vi "Base assingnment EXVI_MS.vi"(5 "BR all info":T11, 6 "Total assembly C":T6 {"Assembly Ratio 2" format="%#_3g"; "Assembly Ratio" format="%#_3g"}, 7 "BC1":cluster{"B region#":i32, "Date":string}, 8 "error in":errorcluster caption="エラー入力", 9 "Selected Raw D":T15, 10 "S New Info and MiN":T26={"Sample Sequence"="GATGATGATGATGATGAT", "Right Read MIN"=6, "Filter P"=0, "STD Type"=enum."Region", "Base Table"=[], "Selection"=enum."10kHz", "noise MAX"=3, "Sample name"=""} {"Base Table"."Value 3" format="%.2g"}, 11 "Filename Path":path) -> (0 "error out":errorcluster caption="エラー出力", 1 "GR data":T21, 2 "Data Histogram":T32(graph), 3 "Table cluster_B":T4, 4 "Ex info":T16)   [LabVIEW 2018]
panel:
  out "Assigned CP Profile plus":T1
  out "Assinged Signal Profile plus":T2
  out "Assigned Time Profile plus":T3
  out "LAP Table":string[][](table) caption="LCP Table"
  out "SOC cluster":T5
  out "Base N info":T7
  out "B Cluster":T8
  out "R std Level":dbl[](array[numeric])
  out "STD Type":enum16{"Region", "Each", "Fixed"}(ring)
  out "BR BL and STD info":T9
  out "BR info":T10
  out "BS Path":T12
  out "BNAL Path":T13
  out "LS Path":T14
  out "B region#":i32
  out "Date":string
  out "Pre File F_Name":string
  out "Base Ex Info":T17
  in  "Data Estimated Info":T18
  out "Base info":T19
  out "Filter P":i32
  out "CP Profile Table P":string[][](table) caption="CP Table"
  out "Time Profile Table P":string[][](table) caption="Time Table"
  out "Signal Profile Table P":string[][](table) caption="表"
  out "Level Composition":string[](array[string])
  out "A level":dbl[](array[numeric])
  out "Filename":string
  out "Time A Table AZ":string[](array[string])
  out "LTP Table":string[][](table) caption="L Time Table for plot"
  out "Filtered Current":dbl[](array[numeric])
  out "Change Point Array":T20
  out "CP Probability":dbl[][](array[numeric])
  out "Time Probability":dbl[][](array[numeric])
  out "Save CV":T22
  out "Table Tag":T23
  out "Table CV":T24
  out "Time A Table Tag":string[](array[string])
  out "CP A Tag AZ":string[](array[string])
  out "Color":u32[](array[numeric])
  out "ASM C":T25
  out "Signal Tag AZ":string[](array[string])
  out "Signal A Table Tag":string[](array[string])
  out "CP A Table Tag":string[](array[string])
  out "R Level":dbl[](array[numeric])
  out "Signal Profile Table":string[][](table) caption="Singla Profile Table"
  in  "Control":enum32{"Set P", "S", "CP", "T"}(tab)
  out "BS Table":string[][](table) caption="Singla Profile Table"
  out "CP Profile Table":string[][](table) caption="CP Table"
  out "Time Profile Table":string[][](table) caption="Time Table"
  in  "I-t":enum32{"Time", "CP", "Assembly", "Plot"}(tab)
  out "Time Graph":cluster{"time":dbl[], "current":dbl[]}[](graph)
  out "Time Graph Profile":cluster{"time":dbl[], dbl[]}[](graph)
  out "Label":T27
  out "CP Graph":cluster{i32[], dbl[]}[](graph)
  out "CP Graph Profile":cluster{i32[], dbl[]}[](graph)
  out "Label 2":T27
  out "std [ratio]":T28={"CP std (ratio)"=200.0, "P std (ratio)"=200.0} {"P std (ratio)" format="%#_3g"; "CP std (ratio)" format="%#_3g"}
  out "Long Assembly":bool[][](array[boolean])
  out "All assembly":bool[][](array[boolean])
  out "assembly C":T29
  out "Signal Number Histogram":cluster{"配列 2":i32[], "配列 5":dbl[]}[](graph)
  out "Right Read MIN":i32=4
  out "LSP Table":string[][](table) caption="Long Singla Profile Table"
  out "Cutted Sample Sequence":string
  out "Base Species (n)":i32
  out "Base (n)":i32
  out "SN [ratio]":T30
  out "Plot Graph":dbl[][](graph)
  out "LCP Table":string[][](table)
  out "F std [pA]":cluster{"CP std (pA)":dbl, "P std (pA)":dbl}={"CP std (pA)"=200.0, "P std (pA)"=200.0} {"P std (pA)" format="%#_13g"; "CP std (pA)" format="%#_13g"}
  out "Relative Data Array":dbl[](array[numeric])
  out "Base Composition":string[](array[string])
  out "Each Base Sequence Info":T31
  out "Sample Sequence":string="GATGATGATGAT"
  in  "time":dbl[](array[numeric])
  in  "current":dbl[](array[numeric])
  out "BS txt":dbl[][](array[numeric])
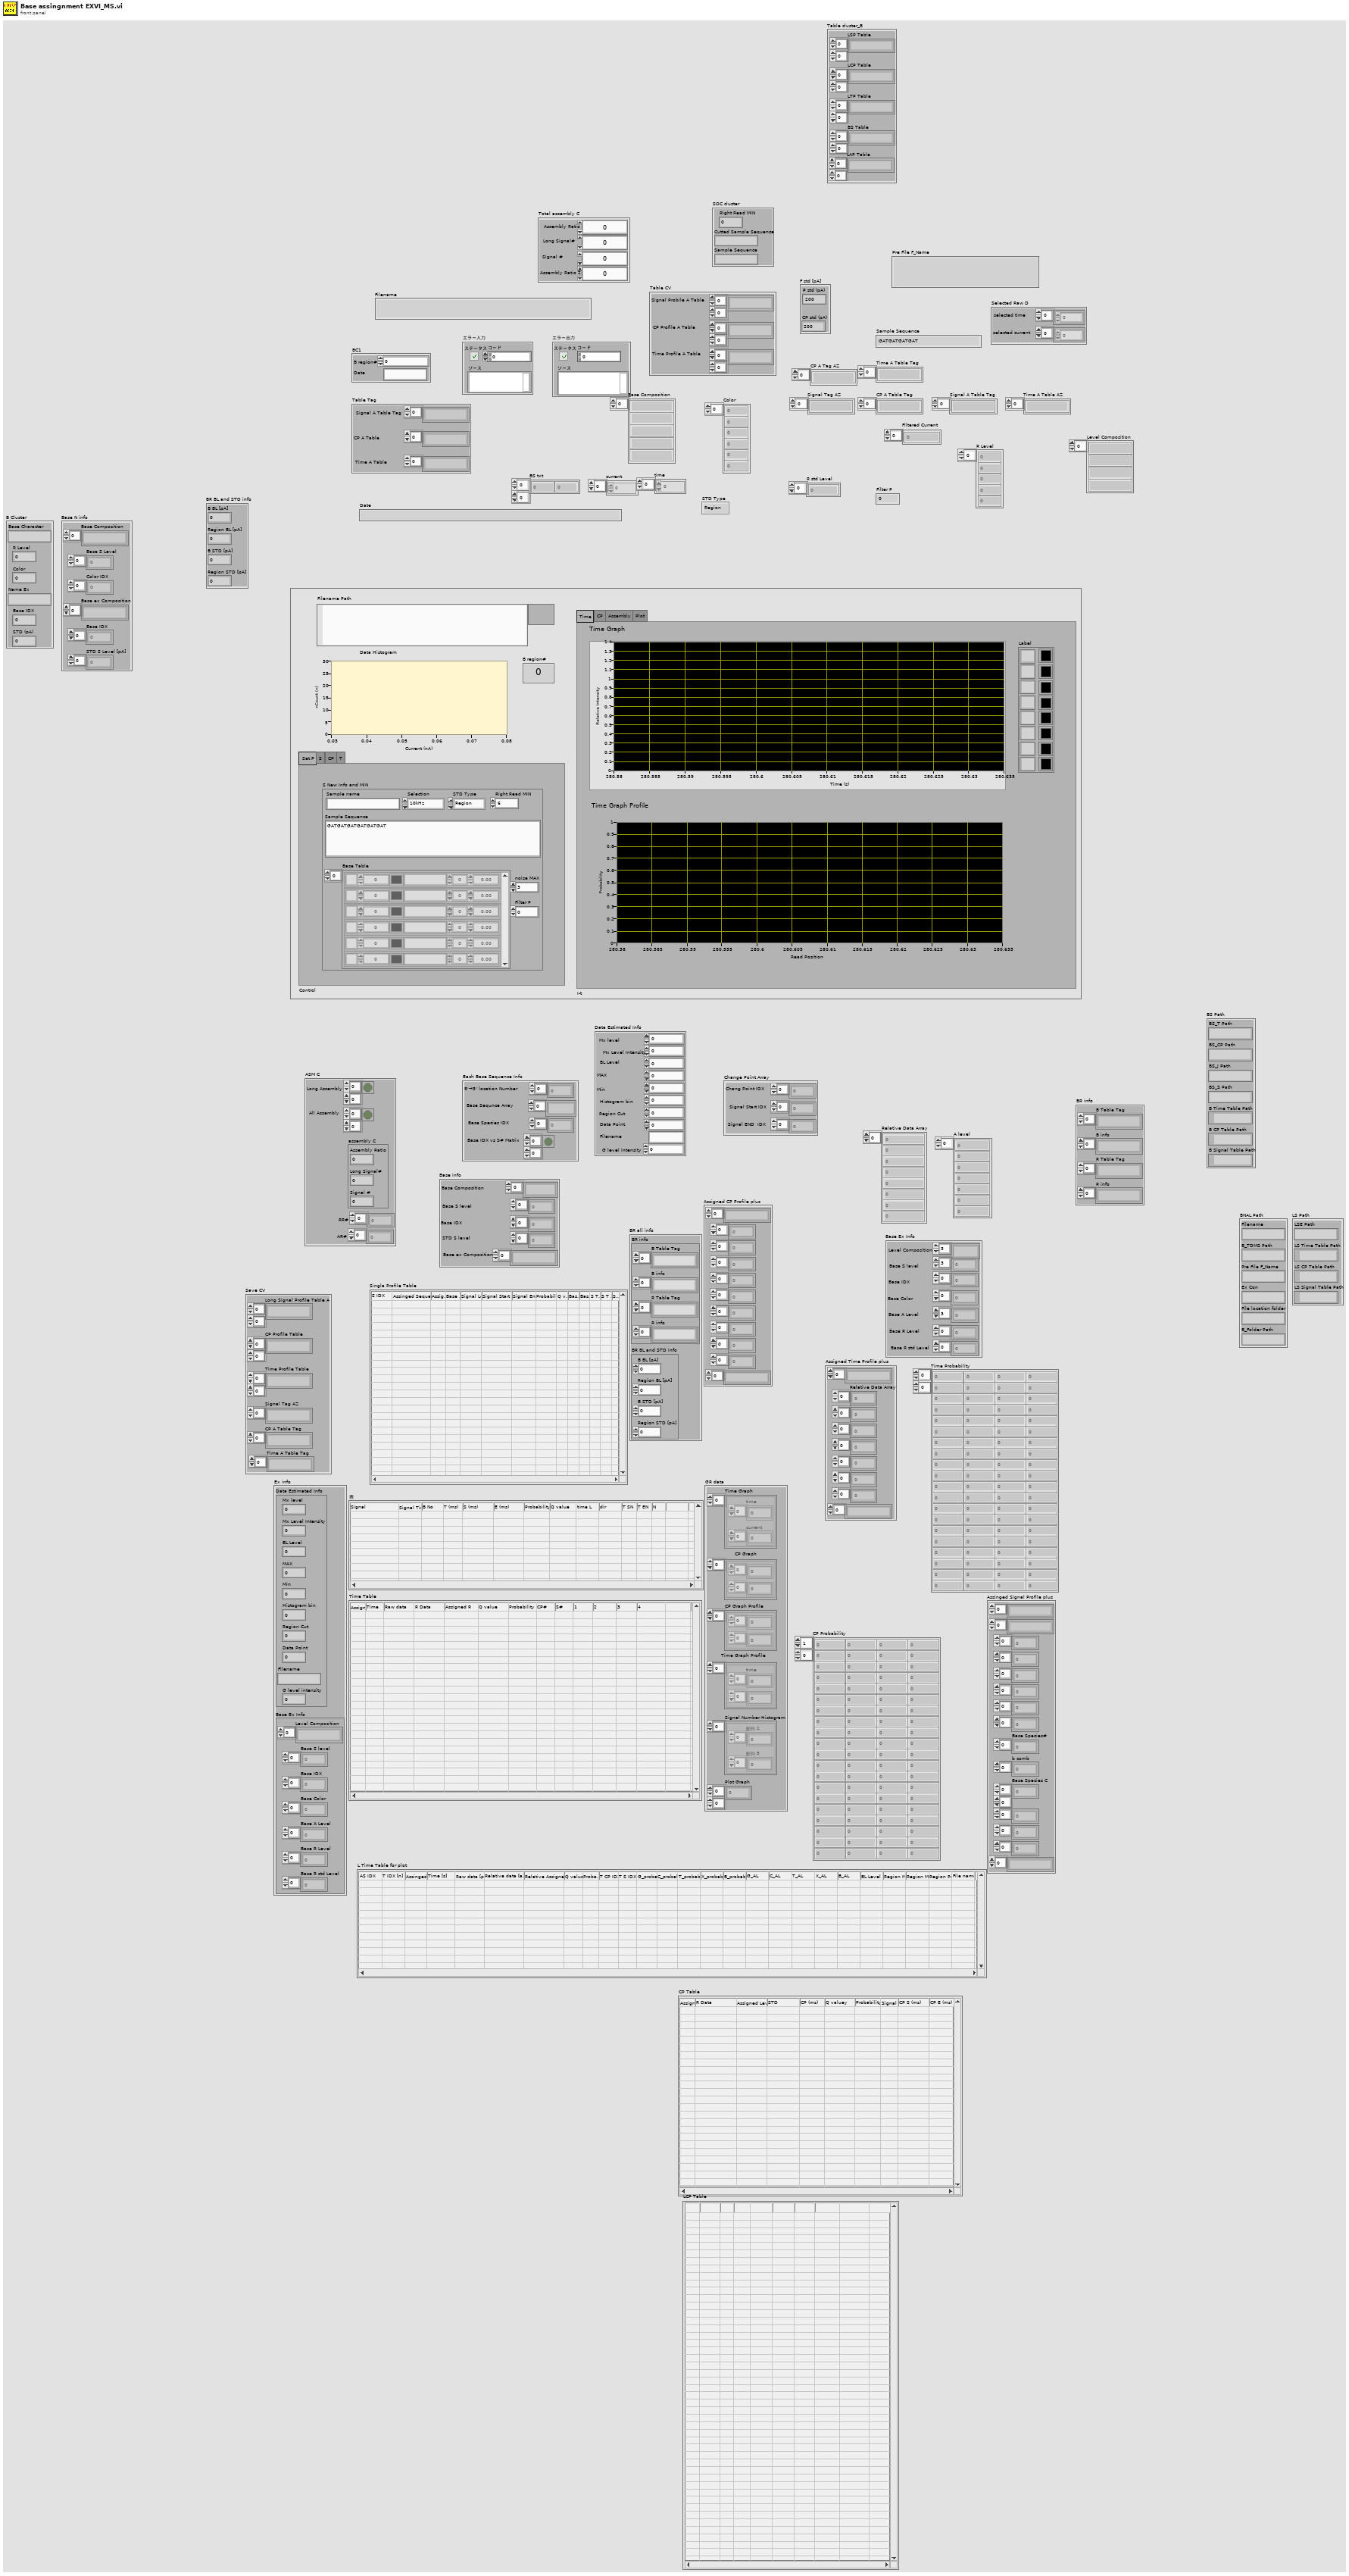
[diagram p1: front panel]
types:
  T1 = cluster{string[], dbl[], dbl[], dbl[], i32[], dbl[], dbl[], i32[], i32[], i32[], string[]}
  T2 = cluster{string[], string[], i32[], i32[], i32[], i32[], dbl[], dbl[], "Base Species#":i16[], "b comb":u32[], "Base Species C":i32[][], i32[], i32[], i32[], string[]}
  T3 = cluster{string[], "Relative Data Array":dbl[], dbl[], dbl[], dbl[], i32[], i32[], i32[], string[]}
  T4 = cluster{"LSP Table":string[][], "LCP Table":string[][], "LTP Table":string[][], "BS Table":string[][], "LAP Table":string[][]}
  T5 = cluster{"Right Read MIN":i32, "Cutted Sample Sequence":string, "Sample Sequence":string}
  T6 = cluster{"Assembly Ratio":dbl, "Long Signal#":i32, "Signal #":i32, "Assembly Ratio 2":dbl}
  T7 = cluster{"Base Composition":string[], "Base S Level":dbl[], "Color IDX":u32[], "Base ex Composition":string[], "Base IDX":i32[], "STD S Level [pA]":dbl[]}
  T8 = cluster{"Base Character":string, "R Level":dbl, "Color":u32, "Name Ex":string, "Base IDX":dbl, "STD (pA)":dbl}
  T9 = cluster{"B BL [pA]":dbl, "Region BL [pA]":dbl, "B STD [pA]":dbl, "Region STD [pA]":dbl}
  T10 = cluster{"B Table Tag":string[], "B info":string[], "R Table Tag":string[], "R info":string[]}
  T11 = cluster{"BR info":cluster{"B Table Tag":string[], "B info":string[], "R Table Tag":string[], "R info":string[]}, "BR BL and STD info":cluster{"B BL [pA]":dbl, "Region BL [pA]":dbl, "B STD [pA]":dbl, "Region STD [pA]":dbl}}
  T12 = cluster{"BS_T Path":string, "BS_CP Path":string, "BS_J Path":string, "BS_S Path":string, "B Time Table Path":path, "B CP Table Path":path, "B Signal Table Path":path}
  T13 = cluster{"Filename":string, "B_TDMS Path":string, "Pre File F_Name":string, "Ex Con":string, "File location folder":string, "B_Folder Path":string}
  T14 = cluster{"LSE Path":string, "LS Time Table Path":path, "LS CP Table Path":path, "LS Signal Table Path":path}
  T15 = cluster{"selected time":dbl[], "selected current":dbl[]}
  T16 = cluster{"Data Estimated Info":cluster{"Mx level":dbl, "Mx Level Intensity":dbl, "BL Level":dbl, "MAX":dbl, "Min":dbl, "Histogram bin":dbl, "Region Cut":dbl, "Data Point":i32, "Filename":string, "G level intensity":dbl}, "Base Ex Info":cluster{"Level Composition":string[], "Base S level":dbl[], "Base IDX":i32[], "Base Color":u32[], "Base A Level":dbl[], "Base R Level":dbl[], "Base R std Level":dbl[]}}
  T17 = cluster{"Level Composition":string[], "Base S level":dbl[], "Base IDX":i32[], "Base Color":u32[], "Base A Level":dbl[], "Base R Level":dbl[], "Base R std Level":dbl[]}
  T18 = cluster{"Mx level":dbl, "Mx Level Intensity":dbl, "BL Level":dbl, "MAX":dbl, "Min":dbl, "Histogram bin":dbl, "Region Cut":dbl, "Data Point":i32, "Filename":string, "G level intensity":dbl}
  T19 = cluster{"Base Composition":string[], "Base S level":dbl[], "Base IDX":i32[], "STD S level":dbl[], "Base ex Composition":string[]}
  T20 = cluster{"Chang Point IDX":i32[], "Signal Start IDX":i32[], "Signal END  IDX":i32[]}
  T21 = cluster{"Time Graph":cluster{"time":dbl[], "current":dbl[]}[], "CP Graph ":cluster{i32[], dbl[]}[], "CP Graph Profile":cluster{i32[], dbl[]}[], "Time Graph Profile":cluster{"time":dbl[], dbl[]}[], "Signal Number Histogram":cluster{"配列 2":i32[], "配列 5":dbl[]}[], "Plot Graph":dbl[][]}
  T22 = cluster{"Long Signal Profile Table A ":string[][], "CP Profile Table":string[][], "Time Profile Table":string[][], "Signal Tag AZ":string[], "CP A Table Tag":string[], "Time A Table Tag":string[]}
  T23 = cluster{"Signal A Table Tag":string[], "CP A Table":string[], "Time A Table":string[]}
  T24 = cluster{"Signal Probile A Table":string[][], "CP Profile A Table":string[][], "Time Profile A Table":string[][]}
  T25 = cluster{"Long Assembly":bool[][], "All Assembly":bool[][], "assembly C":cluster{"Assembly Ratio":dbl, "Long Signal#":i32, "Signal #":i32}, "RR#":i32[], "AR#":i32[]}
  T26 = cluster{"Sample Sequence":string, "Right Read MIN":i32, "Filter P":i32, "STD Type":enum16{"Region", "Each", "Fixed"}, "Base Table":cluster{"Name":string, "Value":dbl, "Color":u32, "Name 2":string, "Value 2":dbl, "Value 3":dbl}[], "Selection":enum16{"10kHz", "100kHz"}, "noise MAX":i32, "Sample name":string}
  T27 = cluster{"カラーボックス":u32, "カラーボックス 4":u32, "カラーボックス 2":u32, "カラーボックス 5":u32, "カラーボックス 3":u32, "カラーボックス 6":u32, "カラーボックス 7":u32, "カラーボックス 8":u32, "B0":string, "B1":string, "B2":string, "B3":string, "B4":string, "B5":string, "B6":string, "B7":string}
  T28 = cluster{"CP std (ratio)":dbl, "P std (ratio)":dbl}
  T29 = cluster{"Assembly Ratio":dbl, "Long Signal#":i32, "Signal #":i32}
  T30 = cluster{"CP S/N ratio":dbl, "T S/N ratio":dbl, "Mx Intensity level [pA]":dbl}
  T31 = cluster{"5'→3' location Number":i32[], "Base Sequnce Array":string[], "Base Species IDX":i32[], "Base IDX vs S# Matrix":bool[][]}
  T32 = cluster{"X Values":dbl[], "Histogram: h(x)":i32[]}
  T33 = cluster{"Name":string, "Value":dbl, "Color":u32, "Name 2":string, "Value 2":dbl, "Value 3":dbl}[]
  T34 = cluster{"B S/N ratio":dbl, "R S/N ratio":dbl, "Mx Intensity level [pA]":dbl}
  T35 = cluster{"CP std [ratio]":dbl, "T std [ratio]":dbl}
  T36 = cluster{"Value":cluster{"Mx level":dbl, "Mx Level Intensity":dbl, "BL Level":dbl, "MAX":dbl, "Min":dbl, "Histogram bin":dbl, "Region Cut":dbl, "Data Point":i32, "Filename":string, "G level intensity":dbl}, "Base Ex Info":cluster{"Level Composition":string[], "Base S level":dbl[], "Base IDX":i32[], "Base Color":u32[], "Base A Level":dbl[], "Base R Level":dbl[], "Base R std Level":dbl[]}}
  T37 = cluster{"Value":string[][], "Value":string[][], "Value":string[][]}
  T38 = cluster{"Value":i32, "Value":string, "Value":string}
  T39 = cluster{"Signal Tag A":string[], "L Signal Tag A":string[]}
  T40 = cluster{"LAP_Table_Tag":string[], "LAP_Table":string[][]}
  T41 = cluster{"Value":string[][], "Value":string[][], "Value":string[][], "Value":string[][], "Value":string[][]}
  T42 = cluster{"Value":cluster{"time":dbl[], "current":dbl[]}[], "Value":cluster{i32[], dbl[]}[], "Value":cluster{i32[], dbl[]}[], "Value":cluster{"time":dbl[], dbl[]}[], "Value":cluster{"配列 2":i32[], "配列 5":dbl[]}[], "Value":dbl[][]}
  T43 = cluster{"Value":string[][], "Value":string[][], "Value":string[][], "Value":string[], "Value":string[], "Value":string[]}
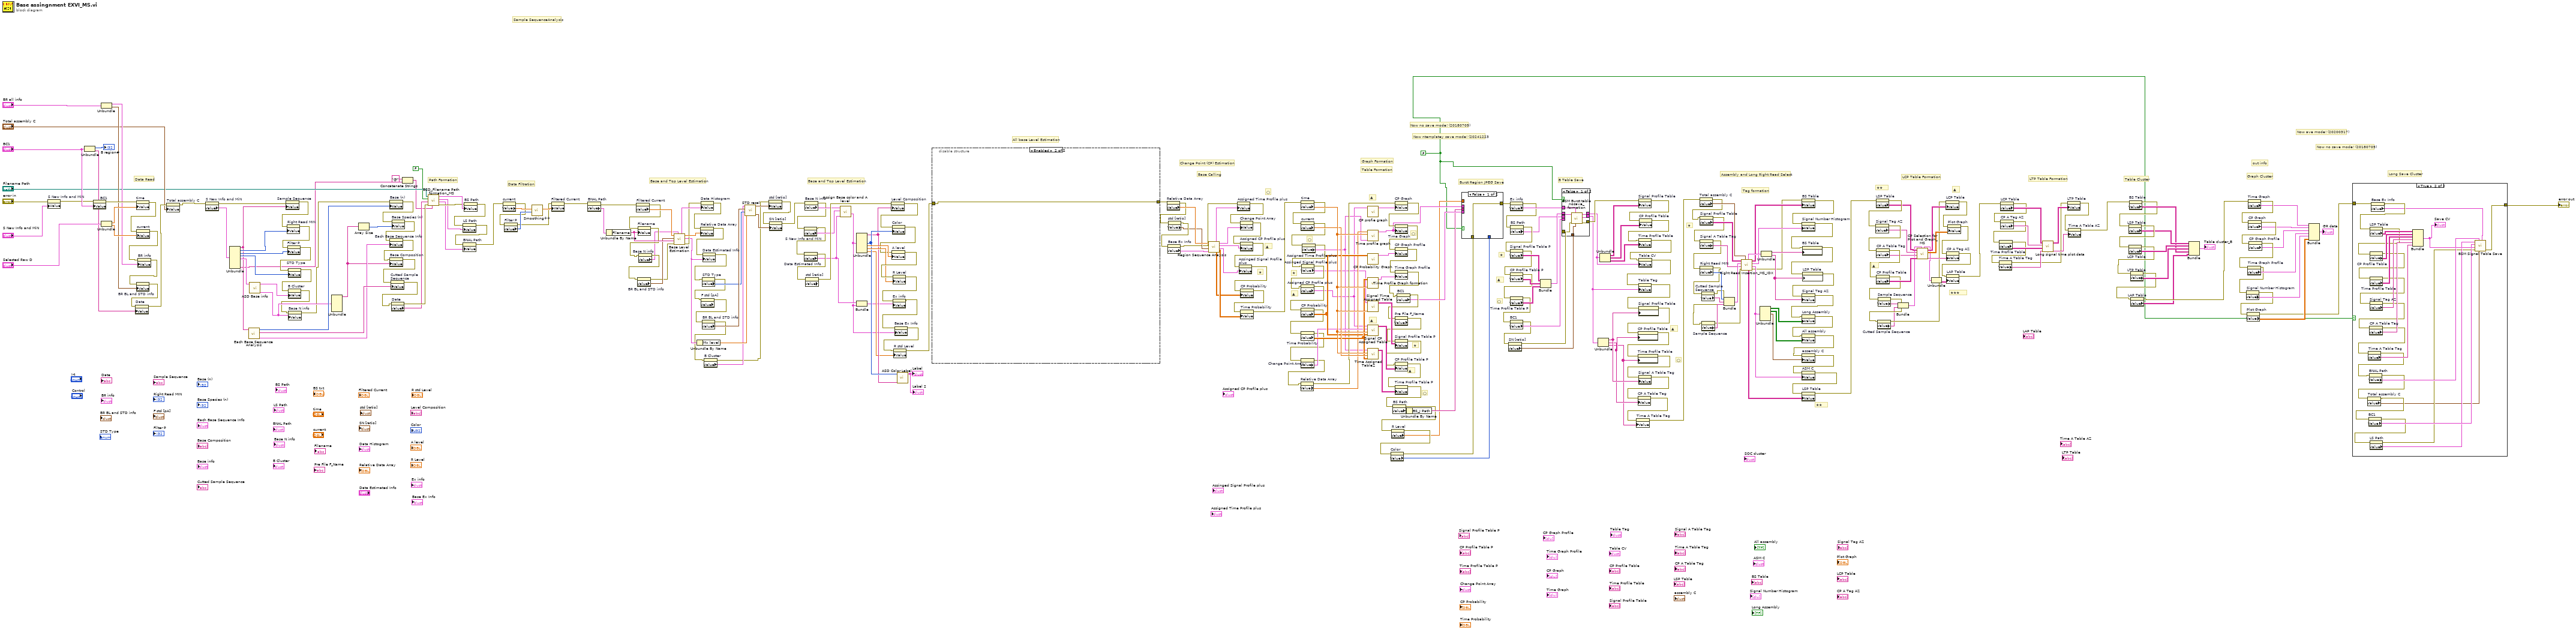
[diagram p0: block diagram]
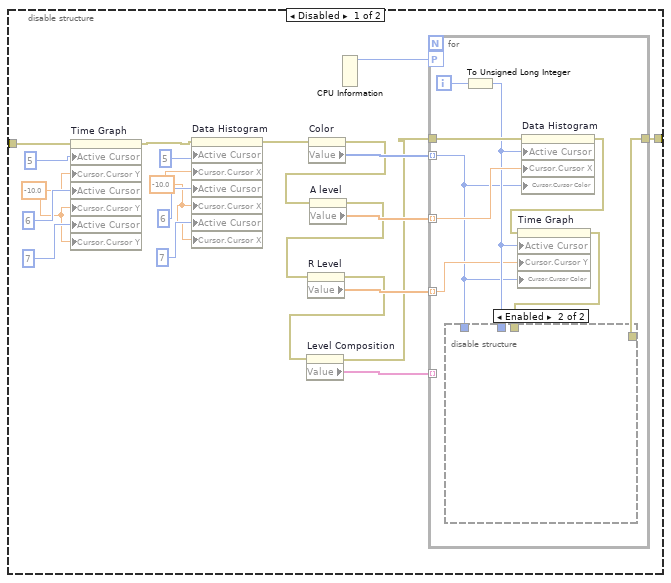
[diagram p2: hidden frame]
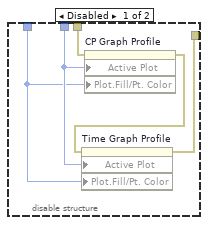
[diagram p3: hidden frame]
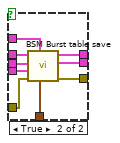
[diagram p5: hidden frame]
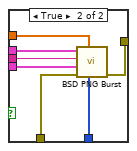
[diagram p6: hidden frame]
diagram:
  w1 = FALSE
  # "Now ntemplatey save mode! (20241223"
  # "▲"
  # "★★★"
  # "★★"
  # "★★"
  # "★"
  # "Tag formation"
  # "〇"
  # "▲"
  # "▲"
  # "▲"
  # "▲"
  # "▲"
  # "▲"
  # "▲"
  # "▲"
  # "〇"
  # "〇"
  # "〇"
  # "★"
  # "★"
  # "★"
  # "〇"
  # "〇"
  # "★"
  # "Now ave mode! (20200317)"
  # "LTP Table Formation"
  # "Now no save mode! (20180709)"
  # "Now no save mode! (20180709)"
  # "Base and Top Level Estimation"
  # "Data Filtration"
  # "out info"
  # "Burst Region JPEG Save"
  # "B Table Save"
  # "Base Calling"
  # "Long Save Cluster"
  # "Table Cluster"
  # "Graph Cluster"
  # "LCP Table Formation"
  # "Assembly and Long Right Read Select"
  # "All base Level Estimation"
  # "Graph Formation"
  # "Table Formation"
  # "Change Point (CP) Estimation"
  # "Path Formation"
  # "Sample SequenceAnalysis"
  # "Base and Top Level Estimation"
  # "Data Read"
  n1 = property on="S New Info and MiN" class="Clust (strict)"(error in="error in", "Value"="S New Info and MiN") -> (error out=w114:errorcluster)  [unwired: 1 in, 1 out]
  n2 = Unbundle("BC1") -> ("B region#"=→"B region#":i32, "Date"=w120:string)
  n3 = property on="BC1" class="Clust (strict)"(error in=w114, "Value"="BC1") -> (error out=w194:errorcluster)  [unwired: 1 in, 1 out]
  n4 = Unbundle("BR all info") -> ("BR info"=w148:T10, "BR BL and STD info"=w149:T9)
  n5 = Unbundle("Selected Raw D") -> ("selected time"=w202:dbl[], "selected current"=w201:dbl[])
  n6 = property on="time" class="Arr (strict)"(error in=w194, "Value"=w202) -> (error out=w306:errorcluster)  [unwired: 1 in, 1 out]
  n7 = property on="current" class="Arr (strict)"(error in=w306, "Value"=w201) -> (error out=w147:errorcluster)  [unwired: 1 in, 1 out]
  n8 = property on="BR info" class="Clust (strict)"(error in=w147, "Value"=w148) -> (error out=w146:errorcluster)  [unwired: 1 in, 1 out]
  n9 = property on="BR BL and STD info" class="Clust (strict)"(error in=w146, "Value"=w149) -> (error out=w119:errorcluster)  [unwired: 1 in, 1 out]
  n10 = property on="Date" class="Str"(error in=w119, "Value"=w120) -> (error out=w80:errorcluster)  [unwired: 1 in, 1 out]
  n11 = property on="Total assembly C" class="Clust (strict)"(error in=w80, "Value"="Total assembly C") -> (error out=w81:errorcluster)  [unwired: 1 in, 1 out]
  n12 = property on="S New Info and MiN" class="Clust (strict)"(error in=w81) -> (error out=w116:errorcluster, "Value"=w113:T26)  [unwired: 1 in, 1 out]
  n13 = Unbundle(w113) -> ("Sample Sequence"=w104:string, "Right Read MIN"=w112:i32, "Filter P"=w111:i32, "STD Type"=w110:enum16{"Region", "Each", "Fixed"}, "Base Table"=w109:T33, "Sample name"=w36:string)  [unwired: 2 out]
  n14 = call "Each Base Sequence Analysis.vi"("Sample Sequence"=w104) -> ("Each Base Sequence Info"=w101:T31, "Cutted Sequence"=w102:string, "Base (n)"=w103:i32)  [unwired: 7 in, 1 out]
  n15 = call "ASD Base info.vi"("Base Table"=w109) -> ("Base N info"=w100:T7, "B Cluster"=w108:T8)  [unwired: 8 in, 1 out]
  n16 = property on="Sample Sequence" class="Str"(error in=w116, "Value"=w104) -> (error out=w212:errorcluster)  [unwired: 1 in, 1 out]
  n17 = property on="Right Read MIN" class="DigNum (strict)"(error in=w212, "Value"=w112) -> (error out=w106:errorcluster)  [unwired: 1 in, 1 out]
  n18 = property on="Filter P" class="DigNum (strict)"(error in=w106, "Value"=w111) -> (error out=w105:errorcluster)  [unwired: 1 in, 1 out]
  n19 = property on="STD Type" class="Enum (strict)"(error in=w105, "Value"=w110) -> (error out=w92:errorcluster)  [unwired: 1 in, 1 out]
  n20 = property on="B Cluster" class="Clust (strict)"(error in=w92, "Value"=w108) -> (error out=w91:errorcluster)  [unwired: 1 in, 1 out]
  n21 = property on="Base N info" class="Clust (strict)"(error in=w91, "Value"=w100) -> (error out=w90:errorcluster)  [unwired: 1 in, 1 out]
  n22 = Unbundle(w100) -> ("Base Composition"=w99:string[])  [unwired: 5 out]
  n23 = Array Size(array=w99) -> (size(s)=w98:i32)
  n24 = property on="Base (n)" class="DigNum (strict)"(error in=w90, "Value"=w103) -> (error out=w227:errorcluster)  [unwired: 1 in, 1 out]
  n25 = property on="Base Species (n)" class="DigNum (strict)"(error in=w227, "Value"=w98) -> (error out=w226:errorcluster)  [unwired: 1 in, 1 out]
  n26 = property on="Each Base Sequence Info" class="Clust (strict)"(error in=w226, "Value"=w101) -> (error out=w225:errorcluster)  [unwired: 1 in, 1 out]
  n27 = property on="Base Composition" class="Arr (strict)"(error in=w225, "Value"=w99) -> (error out=w93:errorcluster)  [unwired: 1 in, 1 out]
  n28 = property on="Cutted Sample Sequence" class="Str"(error in=w93, "Value"=w102) -> (error out=w118:errorcluster)  [unwired: 1 in, 1 out]
  n29 = property on="Date" class="Str"(error in=w118) -> (error out=w44:errorcluster, "Value"=w42:string)  [unwired: 1 in, 1 out]
  n30 = Concatenate Strings("@" ("string"), w36) -> (w35:string)
  n31 = call "BSD_Filename Path formation_MS.vi"("BF_name"=w35, "error in (no error)"=w44, "Date"=w42, "SAVE"=FALSE, "Filename Path"="Filename Path") -> ("error out"=w40:errorcluster, "BNAL Path"=w38:T13, "LS Path"=w39:T14, "BS Path"=w41:T12)  [unwired: 2 in, 1 out]
  n32 = property on="BS Path" class="Clust (strict)"(error in=w40, "Value"=w41) -> (error out=w159:errorcluster)  [unwired: 1 in, 1 out]
  n33 = property on="LS Path" class="Clust (strict)"(error in=w159, "Value"=w39) -> (error out=w196:errorcluster)  [unwired: 1 in, 1 out]
  n34 = property on="BNAL Path" class="Clust (strict)"(error in=w196, "Value"=w38) -> (error out=w168:errorcluster)  [unwired: 1 in, 1 out]
  n35 = property on="current" class="Arr (strict)"(error in=w168) -> (error out=w214:errorcluster, "Value"=w242:dbl[])  [unwired: 1 in, 1 out]
  n36 = property on="Filter P" class="DigNum (strict)"(error in=w214) -> (error out=w213:errorcluster, "Value"=w215:i32)  [unwired: 1 in, 1 out]
  n37 = call "Smoothing++.vi"("+/- Point"=w215, "Y in"=w242) -> ("Y out"=w217:dbl[])  [unwired: 9 in]
  n38 = property on="Filtered Current" class="Arr (strict)"(error in=w213, "Value"=w217) -> (error out=w166:errorcluster)  [unwired: 1 in, 1 out]
  n39 = property on="BNAL Path" class="Clust (strict)"(error in=w166) -> (error out=w165:errorcluster, "Value"=w167:T13)  [unwired: 1 in, 1 out]
  n40 = Unbundle By Name(w167) -> ("Filename"=w164:string)
  n41 = property on="Filtered Current" class="Arr (strict)"(error in=w165) -> (error out=w208:errorcluster, "Value"=w241:dbl[])  [unwired: 1 in, 1 out]
  n42 = property on="Filename" class="Str"(error in=w208, "Value"=w164) -> (error out=w97:errorcluster)  [unwired: 1 in, 1 out]
  n43 = property on="Base N info" class="Clust (strict)"(error in=w97) -> (error out=w96:errorcluster, "Value"=w95:T7)  [unwired: 1 in, 1 out]
  n44 = property on="BR BL and STD info" class="Clust (strict)"(error in=w96) -> (error out=w94:errorcluster, "Value"=w124:T9)  [unwired: 1 in, 1 out]
  n45 = call "Base Level Estimation.vi"("Base N info"=w95, "error in"=w94, "Filename"=w164, "BR BL and STD info"=w124, "Raw data"=w241) -> ("error out"=w218:errorcluster, "Data Estimated Info"=w143:T18, "Relative G Data Array"=w304:dbl[], "Histogram Graph"=w305:T32)  [unwired: 3 in]
  n46 = Unbundle By Name(w143) -> ("Mx level"=w142:dbl)
  n47 = property on="Data Histogram" class="XYGraph (strict)"(error in=w218, "Value"=w305) -> (error out=w303:errorcluster)  [unwired: 1 in, 1 out]
  n48 = property on="Relative Data Array" class="Arr (strict)"(error in=w303, "Value"=w304) -> (error out=w211:errorcluster)  [unwired: 1 in, 1 out]
  n49 = property on="Data Estimated Info" class="Clust (strict)"(error in=w211, "Value"=w143) -> (error out=w136:errorcluster)  [unwired: 1 in, 1 out]
  n50 = property on="STD Type" class="Enum (strict)"(error in=w136) -> (error out=w135:errorcluster, "Value"=w144:enum16{"Region", "Each", "Fixed"})  [unwired: 1 in, 1 out]
  n51 = property on="F std [pA]" class="Clust (strict)" props=["Value"](error in=w135) -> (error out=w134:errorcluster)  [unwired: 1 in, 2 out]
  n52 = property on="BR BL and STD info" class="Clust (strict)"(error in=w134) -> (error out=w83:errorcluster, "Value"=w145:T9)  [unwired: 1 in, 1 out]
  n53 = property on="B Cluster" class="Clust (strict)"(error in=w83) -> (error out=w82:errorcluster, "Value"=w107:T8)  [unwired: 1 in, 1 out]
  n54 = call "STD recal.vi"("Mx Level intensity"=w142, "STD Type"=w144, "BR BL and STD info"=w145, "B Cluster"=w107) -> ("SN [ratio]"=w126:T34, "std [ratio]"=w141:T35)  [unwired: 6 in]
  n55 = property on="std [ratio]" class="Clust (strict)"(error in=w82, "Value"=w141) -> (error out=w125:errorcluster)  [unwired: 1 in, 1 out]
  n56 = property on="SN [ratio]" class="Clust (strict)"(error in=w125, "Value"=w126) -> (error out=w89:errorcluster)  [unwired: 1 in, 1 out]
  n57 = property on="Base N info" class="Clust (strict)"(error in=w89) -> (error out=w85:errorcluster, "Value"=w88:T7)  [unwired: 1 in, 1 out]
  n58 = property on="S New Info and MiN" class="Clust (strict)"(error in=w85) -> (error out=w84:errorcluster, "Value"=w87:T26)  [unwired: 1 in, 1 out]
  n59 = property on="Data Estimated Info" class="Clust (strict)"(error in=w84) -> (error out=w86:errorcluster, "Value"=w26:T18)  [unwired: 1 in, 1 out]
  n60 = property on="std [ratio]" class="Clust (strict)" props=["Value"](error in=w86) -> (error out=w131:errorcluster)  [unwired: 1 in, 2 out]
  n61 = call "Assign Base color and A level.vi"("Data Estimated Info"=w26, "S New Info and MiN"=w87, "Base N info"=w88) -> ("Base Ex Info"=w24:T17)  [unwired: 5 in, 3 out]
  n62 = Unbundle(w24) -> ("Level Composition"=w198:string[], "Base Color"=w199:u32[], "Base A Level"=w207:dbl[], "Base R Level"=w206:dbl[], "Base R std Level"=w133:dbl[])  [unwired: 2 out]
  n63 = Bundle("Value"=w26, "Base Ex Info"=w24) -> (w25:T36)  [unwired: 1 in]
  n64 = property on="Level Composition" class="Arr (strict)"(error in=w131, "Value"=w198) -> (error out=w204:errorcluster)  [unwired: 1 in, 1 out]
  n65 = property on="Color" class="Arr (strict)"(error in=w204, "Value"=w199) -> (error out=w205:errorcluster)  [unwired: 1 in, 1 out]
  n66 = property on="A level" class="Arr (strict)"(error in=w205, "Value"=w207) -> (error out=w224:errorcluster)  [unwired: 1 in, 1 out]
  n67 = property on="R Level" class="Arr (strict)"(error in=w224, "Value"=w206) -> (error out=w27:errorcluster)  [unwired: 1 in, 1 out]
  n68 = property on="Ex info" class="Clust (strict)"("Value"=w25) -> ()  [unwired: 2 in, 2 out]
  n69 = property on="Base Ex Info" class="Clust (strict)"(error in=w27, "Value"=w24) -> (error out=w132:errorcluster)  [unwired: 1 in, 1 out]
  n70 = property on="R std Level" class="Arr (strict)"(error in=w132, "Value"=w133) -> (error out=w130:errorcluster)  [unwired: 1 in, 1 out]
  n71 = call "ASD Color Label.vi"("Level Composition"=w198, "Color"=w199) -> ("Label"=→"Label" →"Label 2":T27)  [unwired: 9 in]
  n72 = disable-structure shown="Enabled" {
    disable-tunnel: [w319 w342] -> w216
    disable-tunnel: w130 -> [w309 w342]
    frame Disabled {
      w313 = -10.0 ("カーソル.カーソル位置:カーソルX")
      w311 = -10.0 ("カーソル.カーソル位置:カーソルX")
      n73 = property on="Time Graph" class="XYGraph (strict)"(error in=w309, "Active Cursor"=u32 5 ("アクティブカーソル"), "Cursor.Cursor Y"=w313, "Active Cursor"=u32 6 ("アクティブカーソル"), "Cursor.Cursor Y"=w313, "Active Cursor"=u32 7 ("アクティブカーソル"), "Cursor.Cursor Y"=w313) -> (error out=w308:errorcluster)  [unwired: 1 in, 1 out]
      n74 = property on="Data Histogram" class="XYGraph (strict)"(error in=w308, "Active Cursor"=u32 5 ("アクティブカーソル"), "Cursor.Cursor X"=w311, "Active Cursor"=u32 6 ("アクティブカーソル"), "Cursor.Cursor X"=w311, "Active Cursor"=u32 7 ("アクティブカーソル"), "Cursor.Cursor X"=w311) -> (error out=w307:errorcluster)  [unwired: 1 in, 1 out]
      n75 = property on="Color" class="Arr (strict)"(error in=w307) -> (error out=w323:errorcluster, "Value"=w325:u32[])  [unwired: 1 in, 1 out]
      n76 = property on="A level" class="Arr (strict)"(error in=w323) -> (error out=w322:errorcluster, "Value"=w326:dbl[])  [unwired: 1 in, 1 out]
      n77 = property on="R Level" class="Arr (strict)"(error in=w322) -> (error out=w321:errorcluster, "Value"=w327:dbl[])  [unwired: 1 in, 1 out]
      n78 = property on="Level Composition" class="Arr (strict)"(error in=w321) -> (error out=w320:errorcluster, "Value"=w324:string[])  [unwired: 1 in, 1 out]
      n79 = CPU Information() -> (4:w310:i32)  [unwired: 3 out]
      n80 = for {
        workers-P: w310 -> [_]
        tunnel: w326 -> [w335] mode=indexing
        tunnel: w325 -> [w328] mode=indexing
        tunnel: w320 -> [w334]
        tunnel: [w329] -> w319
        tunnel: w324 -> [_] mode=indexing
        tunnel: w327 -> [w332] mode=indexing
        i -> [w336]
        n81 = To Unsigned Long Integer(number=w336) -> (unsigned 32bit integer=w333:u32)
        n82 = property on="Data Histogram" class="XYGraph (strict)"(error in=w334, "Active Cursor"=w333, "Cursor.Cursor X"=w335, "Cursor.Cursor Color"=w328) -> (error out=w331:errorcluster)  [unwired: 1 in, 1 out]
        n83 = property on="Time Graph" class="XYGraph (strict)"(error in=w331, "Active Cursor"=w333, "Cursor.Cursor Y"=w332, "Cursor.Cursor Color"=w328) -> (error out=w330:errorcluster)  [unwired: 1 in, 1 out]
        n84 = disable-structure shown="Enabled" {
          disable-tunnel: w333 -> [w341 _]
          disable-tunnel: w330 -> [w340 _]
          disable-tunnel: [w338 _] -> w329
          disable-tunnel: w328 -> [w337 _]
          frame Disabled {
            n85 = property on="CP Graph Profile" class="XYGraph (strict)"(error in=w340, "Active Plot"=w341, "Plot.Fill/Pt. Color"=w337) -> (error out=w339:errorcluster)  [unwired: 1 in, 1 out]
            n86 = property on="Time Graph Profile" class="XYGraph (strict)"(error in=w339, "Active Plot"=w341, "Plot.Fill/Pt. Color"=w337) -> (error out=w338:errorcluster)  [unwired: 1 in, 1 out]
          }
          frame Enabled {
          }
        }
      }
    }
    frame Enabled {
    }
  }
  n87 = property on="Relative Data Array" class="Arr (strict)"(error in=w216) -> (error out=w140:errorcluster, "Value"=w302:dbl[])  [unwired: 1 in, 1 out]
  n88 = property on="std [ratio]" class="Clust (strict)"(error in=w140) -> (error out=w139:errorcluster, "Value"=w138:T28)  [unwired: 1 in, 1 out]
  n89 = property on="Base Ex Info" class="Clust (strict)"(error in=w139) -> (error out=w16:errorcluster, "Value"=w209:T17)  [unwired: 1 in, 1 out]
  n90 = call "Region Sequence Anaysis.vi"("Base Ex Info"=w209, "std"=w138, "Relative Data Array"=w302) -> ("Assinged Signal Profile plus"=w13:T2, "Assigned CP Profile plus"=w6:T1, "Change Point Array"=w248:T20, "CP Probability"=w249:dbl[][], "Assigned Time Profile plus"=w14:T3, "Time Probability"=w252:dbl[][])  [unwired: 2 in, 1 out]
  n91 = property on="Assigned Time Profile plus" class="Clust (strict)"(error in=w16, "Value"=w14) -> (error out=w15:errorcluster)  [unwired: 1 in, 1 out]
  n92 = property on="Change Point Array" class="Clust (strict)"(error in=w15, "Value"=w248) -> (error out=w8:errorcluster)  [unwired: 1 in, 1 out]
  n93 = property on="Assigned CP Profile plus" class="Clust (strict)"(error in=w8, "Value"=w6) -> (error out=w7:errorcluster)  [unwired: 1 in, 1 out]
  n94 = property on="Assinged Signal Profile plus" class="Clust (strict)"(error in=w7, "Value"=w13) -> (error out=w12:errorcluster)  [unwired: 1 in, 1 out]
  n95 = property on="CP Probability" class="Arr (strict)"(error in=w12, "Value"=w249) -> (error out=w244:errorcluster)  [unwired: 1 in, 1 out]
  n96 = property on="Time Probability" class="Arr (strict)"(error in=w244, "Value"=w252) -> (error out=w243:errorcluster)  [unwired: 1 in, 1 out]
  n97 = property on="time" class="Arr (strict)"(error in=w243) -> (error out=w288:errorcluster, "Value"=w301:dbl[])  [unwired: 1 in, 1 out]
  n98 = property on="current" class="Arr (strict)"(error in=w288) -> (error out=w11:errorcluster, "Value"=w289:dbl[])  [unwired: 1 in, 1 out]
  n99 = property on="Assigned Time Profile plus" class="Clust (strict)"(error in=w11) -> (error out=w9:errorcluster, "Value"=w10:T3)  [unwired: 1 in, 1 out]
  n100 = property on="Assinged Signal Profile plus" class="Clust (strict)"(error in=w9) -> (error out=w5:errorcluster, "Value"=w3:T2)  [unwired: 1 in, 1 out]
  n101 = property on="Assigned CP Profile plus" class="Clust (strict)"(error in=w5) -> (error out=w4:errorcluster, "Value"=w2:T1)  [unwired: 1 in, 1 out]
  n102 = property on="CP Probability" class="Arr (strict)"(error in=w4) -> (error out=w246:errorcluster, "Value"=w250:dbl[][])  [unwired: 1 in, 1 out]
  n103 = property on="Time Probability" class="Arr (strict)"(error in=w246) -> (error out=w245:errorcluster, "Value"=w251:dbl[][])  [unwired: 1 in, 1 out]
  n104 = property on="Change Point Array" class="Clust (strict)"(error in=w245) -> (error out=w128:errorcluster, "Value"=w247:T20)  [unwired: 1 in, 1 out]
  n105 = property on="Relative Data Array" class="Arr (strict)"(error in=w128) -> (error out=w127:errorcluster, "Value"=w129:dbl[])  [unwired: 1 in, 1 out]
  n106 = call "CP profie graph.vi"("Assigned CP Profile plus"=w2) -> ("CP Graph Profile"=w228:cluster{i32[], dbl[]}[])  [unwired: 10 in]
  n107 = call "Time profile graph.vi"("Assigned Time Profile plus"=w10, "time"=w301, "Relative Data Array"=w129) -> ("Signal Time Graph"=w195:cluster{"time":dbl[], "current":dbl[]}[])  [unwired: 8 in]
  n108 = call "CP Probability Graph.vi"("CP Probability"=w250) -> ("CP Graph Profile"=w256:cluster{i32[], dbl[]}[])  [unwired: 10 in]
  n109 = call "Time Profile Graph formation.vi"("time"=w301, "CP Probability"=w251) -> ("Time Profile Graph"=w257:cluster{"time":dbl[], dbl[]}[])  [unwired: 9 in]
  n110 = call "Signal Time Assigned Table.vi"("time"=w301, "Assinged Signal Profile plus"=w3) -> ("Signal Profile Table"=w223:string[][])  [unwired: 9 in]
  n111 = call "Signal CP Assigned Table.vi"("CP Probability"=w250, "time"=w301, "Change Point Array"=w247, "Assigned CP Profile plus"=w2) -> ("CP Profile Table"=w221:string[][])  [unwired: 7 in]
  n112 = call "Time Assigned TableZ.vi"("Time Probability"=w251, "current"=w289, "time"=w301, "Assigned Time Profile plus"=w10) -> ("Time Profile Table P"=w222:string[][])  [unwired: 7 in]
  n113 = property on="CP Graph" class="XYGraph (strict)"(error in=w127, "Value"=w228) -> (error out=w255:errorcluster)  [unwired: 1 in, 1 out]
  n114 = property on="Time Graph" class="XYGraph (strict)"(error in=w255, "Value"=w195) -> (error out=w254:errorcluster)  [unwired: 1 in, 1 out]
  n115 = property on="CP Graph Profile" class="XYGraph (strict)"(error in=w254, "Value"=w256) -> (error out=w253:errorcluster)  [unwired: 1 in, 1 out]
  n116 = property on="Time Graph Profile" class="XYGraph (strict)"(error in=w253, "Value"=w257) -> (error out=w192:errorcluster)  [unwired: 1 in, 1 out]
  n117 = property on="BC1" class="Clust (strict)"(error in=w192) -> (error out=w191:errorcluster, "Value"=w190:cluster{"B region#":i32, "Date":string})  [unwired: 1 in, 1 out]
  n118 = property on="Pre File F_Name" class="Str" props=["Value"](error in=w191) -> (error out=w200:errorcluster)  [unwired: 1 in, 2 out]
  n119 = property on="Signal Profile Table P" class="Tbl (strict)"(error in=w200, "Value"=w223) -> (error out=w220:errorcluster)  [unwired: 1 in, 1 out]
  n120 = property on="CP Profile Table P" class="Tbl (strict)"(error in=w220, "Value"=w221) -> (error out=w219:errorcluster)  [unwired: 1 in, 1 out]
  n121 = property on="Time Profile Table P" class="Tbl (strict)"(error in=w219, "Value"=w222) -> (error out=w158:errorcluster)  [unwired: 1 in, 1 out]
  n122 = property on="BS Path" class="Clust (strict)"(error in=w158) -> (error out=w157:errorcluster, "Value"=w156:T12)  [unwired: 1 in, 1 out]
  n123 = property on="R Level" class="Arr (strict)"(error in=w157) -> (error out=w163:errorcluster, "Value"=w160:dbl[])  [unwired: 1 in, 1 out]
  n124 = property on="Color" class="Arr (strict)"(error in=w163) -> (error out=w162:errorcluster, "Value"=w161:u32[])  [unwired: 1 in, 1 out]
  n125 = Unbundle By Name(w156) -> ("BS_J Path"=w189:string)
  n126 = case shown="False" w1 {
    tunnel: w195 -> [_ w350]
    tunnel: w190 -> [_ w349]
    tunnel: w189 -> [_ w348]
    tunnel: [w343 w347] -> w173
    tunnel: w162 -> [w343 w346]
    tunnel: w161 -> [_ w345]
    tunnel: w160 -> [_ w344]
    frame False {
    }
    frame True {
      n127 = call "BSD PNG Burst.vi"("Color"=w345, "R Level"=w344, "error in"=w346, "BC1"=w349, "BSE path"=w348, "Time Graph"=w350) -> ("error out"=w347:errorcluster)  [unwired: 5 in]
    }
  }
  n128 = property on="Ex info" class="Clust (strict)"(error in=w173) -> (error out=w155:errorcluster, "Value"=w176:T16)  [unwired: 1 in, 1 out]
  n129 = property on="BS Path" class="Clust (strict)"(error in=w155) -> (error out=w154:errorcluster, "Value"=w153:T12)  [unwired: 1 in, 1 out]
  n130 = property on="Signal Profile Table P" class="Tbl (strict)"(error in=w154) -> (error out=w184:errorcluster, "Value"=w187:string[][])  [unwired: 1 in, 1 out]
  n131 = property on="CP Profile Table P" class="Tbl (strict)"(error in=w184) -> (error out=w183:errorcluster, "Value"=w186:string[][])  [unwired: 1 in, 1 out]
  n132 = property on="Time Profile Table P" class="Tbl (strict)"(error in=w183) -> (error out=w182:errorcluster, "Value"=w185:string[][])  [unwired: 1 in, 1 out]
  n133 = property on="BC1" class="Clust (strict)"(error in=w182) -> (error out=w122:errorcluster, "Value"=w175:cluster{"B region#":i32, "Date":string})  [unwired: 1 in, 1 out]
  n134 = property on="SN [ratio]" class="Clust (strict)"(error in=w122) -> (error out=w121:errorcluster, "Value"=w123:T30)  [unwired: 1 in, 1 out]
  n135 = Bundle("Value"=w187, "Value"=w186, "Value"=w185) -> (w181:T37)  [unwired: 1 in]
  n136 = case shown="False" w1 {
    tunnel: [w355 w366] -> w188
    tunnel: w181 -> [w351 w365]
    tunnel: [w354 w364] -> w177
    tunnel: w176 -> [w357 w363]
    tunnel: w175 -> [_ w362]
    tunnel: [w353 w361] -> w174
    tunnel: w153 -> [_ w360]
    tunnel: w123 -> [w352 w359]
    tunnel: w121 -> [w356 w358]
    frame False {
      n137 = call "BSM Burst table nosave_formation.vi"("SN [ratio]"=w352, "Ex info"=w357, "error in"=w356, "Table CP"=w351) -> ("error out"=w355:errorcluster, "Table Tag"=w353:T23, "Table CV"=w354:T24)  [unwired: 5 in]
    }
    frame True {
      n138 = call "BSM Burst table save.vi"("SN [ratio]"=w359, "Ex info"=w363, "error in"=w358, "BC1"=w362, "BS Path"=w360, "Table CP"=w365) -> ("error out"=w366:errorcluster, "Table Tag"=w361:T23, "Table CV"=w364:T24)  [unwired: 3 in]
    }
  }
  n139 = Unbundle(w174) -> ("Signal A Table Tag"=w172:string[], "CP A Table"=w171:string[], "Time A Table"=w170:string[])
  n140 = Unbundle(w177) -> ("Signal Probile A Table"=w180:string[][], "CP Profile A Table"=w179:string[][], "Time Profile A Table"=w178:string[][])
  n141 = property on="Signal Profile Table" class="Tbl (strict)"(error in=w188, "Value"=w180) -> (error out=w262:errorcluster)  [unwired: 1 in, 1 out]
  n142 = property on="CP Profile Table" class="Tbl (strict)"(error in=w262, "Value"=w179) -> (error out=w261:errorcluster)  [unwired: 1 in, 1 out]
  n143 = property on="Time Profile Table" class="Tbl (strict)"(error in=w261, "Value"=w178) -> (error out=w260:errorcluster)  [unwired: 1 in, 1 out]
  n144 = property on="Table CV" class="Clust (strict)"(error in=w260, "Value"=w177) -> (error out=w259:errorcluster)  [unwired: 1 in, 1 out]
  n145 = property on="Table Tag" class="Clust (strict)"(error in=w259, "Value"=w174) -> (error out=w258:errorcluster)  [unwired: 1 in, 1 out]
  n146 = property on="Signal Profile Table" class="Tbl (strict)"(error in=w258, "Column Headers[]"=w172) -> (error out=w299:errorcluster)  [unwired: 1 in, 1 out]
  n147 = property on="CP Profile Table" class="Tbl (strict)"(error in=w299, "Column Headers[]"=w171) -> (error out=w300:errorcluster)  [unwired: 1 in, 1 out]
  n148 = property on="Time Profile Table" class="Tbl (strict)"(error in=w300, "Column Headers[]"=w170) -> (error out=w279:errorcluster)  [unwired: 1 in, 1 out]
  n149 = property on="Signal A Table Tag" class="Arr (strict)"(error in=w279, "Value"=w172) -> (error out=w278:errorcluster)  [unwired: 1 in, 1 out]
  n150 = property on="CP A Table Tag" class="Arr (strict)"(error in=w278, "Value"=w171) -> (error out=w277:errorcluster)  [unwired: 1 in, 1 out]
  n151 = property on="Time A Table Tag" class="Arr (strict)"(error in=w277, "Value"=w170) -> (error out=w33:errorcluster)  [unwired: 1 in, 1 out]
  n152 = property on="Total assembly C" class="Clust (strict)"(error in=w33) -> (error out=w32:errorcluster, "Value"=w65:T6)  [unwired: 1 in, 1 out]
  n153 = property on="Signal Profile Table" class="Tbl (strict)"(error in=w32) -> (error out=w31:errorcluster, "Value"=w75:string[][])  [unwired: 1 in, 1 out]
  n154 = property on="Signal A Table Tag" class="Arr (strict)"(error in=w31) -> (error out=w30:errorcluster, "Value"=w73:string[])  [unwired: 1 in, 1 out]
  n155 = property on="Right Read MIN" class="DigNum (strict)"(error in=w30) -> (error out=w29:errorcluster, "Value"=w78:i32)  [unwired: 1 in, 1 out]
  n156 = property on="Cutted Sample Sequence" class="Str"(error in=w29) -> (error out=w28:errorcluster, "Value"=w77:string)  [unwired: 1 in, 1 out]
  n157 = property on="Sample Sequence" class="Str"(error in=w28) -> (error out=w72:errorcluster, "Value"=w76:string)  [unwired: 1 in, 1 out]
  n158 = Bundle("Value"=w78, "Value"=w77, "Value"=w76) -> (w74:T38)  [unwired: 1 in]
  n159 = call "Right Read Insertion_MS_IDX.vi"("Total assembly C"=w65, "error in"=w72, "Signal Tag"=w73, "SOC cluster"=w74, "Signal Profile Table"=w75) -> ("error out"=w67:errorcluster, "ASM C"=w68:T25, "Signal Number Histogram"=w69:cluster{"配列 2":i32[], "配列 5":dbl[]}[], "BS Table"=w70:string[][], "LSP Table"=w66:string[][], "LSS Tag"=w71:T39)  [unwired: 1 in]
  n160 = Unbundle(w68) -> ("Long Assembly"=w271:bool[][], "All Assembly"=w272:bool[][], "assembly C"=w273:T29)  [unwired: 2 out]
  n161 = Unbundle(w71) -> ("Signal Tag A"=w152:string[], "L Signal Tag A"=w151:string[])
  n162 = property on="BS Table" class="Tbl (strict)"(error in=w67, "Value"=w70) -> (error out=w270:errorcluster)  [unwired: 1 in, 1 out]
  n163 = property on="Signal Number Histogram" class="XYGraph (strict)"(error in=w270, "Value"=w69) -> (error out=w269:errorcluster)  [unwired: 1 in, 1 out]
  n164 = property on="BS Table" class="Tbl (strict)"(error in=w269, "Column Headers[]"=w152) -> (error out=w298:errorcluster)  [unwired: 1 in, 1 out]
  n165 = property on="LSP Table" class="Tbl (strict)"(error in=w298, "Column Headers[]"=w151) -> (error out=w282:errorcluster)  [unwired: 1 in, 1 out]
  n166 = property on="Signal Tag AZ" class="Arr (strict)"(error in=w282, "Value"=w151) -> (error out=w268:errorcluster)  [unwired: 1 in, 1 out]
  n167 = property on="Long Assembly" class="Arr (strict)"(error in=w268, "Value"=w271) -> (error out=w267:errorcluster)  [unwired: 1 in, 1 out]
  n168 = property on="All assembly" class="Arr (strict)"(error in=w267, "Value"=w272) -> (error out=w266:errorcluster)  [unwired: 1 in, 1 out]
  n169 = property on="assembly C" class="Clust (strict)"(error in=w266, "Value"=w273) -> (error out=w265:errorcluster)  [unwired: 1 in, 1 out]
  n170 = property on="ASM C" class="Clust (strict)"(error in=w265, "Value"=w68) -> (error out=w264:errorcluster)  [unwired: 1 in, 1 out]
  n171 = property on="LSP Table" class="Tbl (strict)"(error in=w264, "Value"=w66) -> (error out=w263:errorcluster)  [unwired: 1 in, 1 out]
  n172 = property on="LSP Table" class="Tbl (strict)"(error in=w263) -> (error out=w276:errorcluster, "Value"=w64:string[][])  [unwired: 1 in, 1 out]
  n173 = property on="Signal Tag AZ" class="Arr (strict)"(error in=w276) -> (error out=w275:errorcluster, "Value"=w63:string[])  [unwired: 1 in, 1 out]
  n174 = property on="CP A Table Tag" class="Arr (strict)"(error in=w275) -> (error out=w274:errorcluster, "Value"=w62:string[])  [unwired: 1 in, 1 out]
  n175 = property on="CP Profile Table" class="Tbl (strict)"(error in=w274) -> (error out=w57:errorcluster, "Value"=w61:string[][])  [unwired: 1 in, 1 out]
  n176 = property on="Sample Sequence" class="Str"(error in=w57) -> (error out=w56:errorcluster, "Value"=w54:string)  [unwired: 1 in, 1 out]
  n177 = property on="Cutted Sample Sequence" class="Str"(error in=w56) -> (error out=w55:errorcluster, "Value"=w53:string)  [unwired: 1 in, 1 out]
  n178 = Bundle("Value"=w54, "Value"=w53) -> (w52:cluster{"Value":string, "Value":string})  [unwired: 1 in]
  n179 = call "CP Selection for Plot and Graph_MS.vi"("Sample cluster"=w52, "CP Profile Table"=w61, "CP A Tag"=w62, "Signal Tag AZ"=w63, "Long Signal Profile Table A"=w64) -> ("CP A Tag AZ"=w58:string[], "Plot Graph"=w59:dbl[][], "LCP Table"=w60:string[][], "LAP"=w23:T40)  [unwired: 2 in, 1 out]
  n180 = Unbundle(w23) -> ("LAP_Table"=w22:string[][])  [unwired: 1 out]
  n181 = property on="LCP Table" class="Tbl (strict)"(error in=w55, "Value"=w60) -> (error out=w281:errorcluster)  [unwired: 1 in, 1 out]
  n182 = property on="Plot Graph" class="IntGraph (strict)"(error in=w281, "Value"=w59) -> (error out=w280:errorcluster)  [unwired: 1 in, 1 out]
  n183 = property on="CP A Tag AZ" class="Arr (strict)"(error in=w280, "Value"=w58) -> (error out=w21:errorcluster)  [unwired: 1 in, 1 out]
  n184 = property on="LAP Table" class="Tbl (strict)"(error in=w21, "Value"=w22) -> (error out=w20:errorcluster)  [unwired: 1 in, 1 out]
  n185 = property on="LCP Table" class="Tbl (strict)"(error in=w20) -> (error out=w236:errorcluster, "Value"=w238:string[][])  [unwired: 1 in, 1 out]
  n186 = property on="CP A Tag AZ" class="Arr (strict)"(error in=w236) -> (error out=w235:errorcluster, "Value"=w237:string[])  [unwired: 1 in, 1 out]
  n187 = property on="Time Profile Table" class="Tbl (strict)"(error in=w235) -> (error out=w234:errorcluster, "Value"=w239:string[][])  [unwired: 1 in, 1 out]
  n188 = property on="Time A Table Tag" class="Arr (strict)"(error in=w234) -> (error out=w231:errorcluster, "Value"=w240:string[])  [unwired: 1 in, 1 out]
  n189 = call "Long signal time plot data.vi"("Time A Table Tag"=w240, "Time Profile Table"=w239, "CP A Tag AZ"=w237, "CP Profile Table for plot"=w238) -> ("Time A Table AZ"=w232:string[], "L Time Profile Table for plot"=w233:string[][])  [unwired: 6 in]
  n190 = property on="LTP Table" class="Tbl (strict)"(error in=w231, "Value"=w233) -> (error out=w230:errorcluster)  [unwired: 1 in, 1 out]
  n191 = property on="Time A Table AZ" class="Arr (strict)"(error in=w230, "Value"=w232) -> (error out=w229:errorcluster)  [unwired: 1 in, 1 out]
  n192 = property on="BS Table" class="Tbl (strict)"(error in=w229) -> (error out=w46:errorcluster, "Value"=w47:string[][])  [unwired: 1 in, 1 out]
  n193 = property on="LSP Table" class="Tbl (strict)"(error in=w46) -> (error out=w287:errorcluster, "Value"=w50:string[][])  [unwired: 1 in, 1 out]
  n194 = property on="LCP Table" class="Tbl (strict)"(error in=w287) -> (error out=w45:errorcluster, "Value"=w49:string[][])  [unwired: 1 in, 1 out]
  n195 = property on="LTP Table" class="Tbl (strict)"(error in=w45) -> (error out=w19:errorcluster, "Value"=w48:string[][])  [unwired: 1 in, 1 out]
  n196 = property on="LAP Table" class="Tbl (strict)"(error in=w19) -> (error out=w18:errorcluster, "Value"=w17:string[][])  [unwired: 1 in, 1 out]
  n197 = Bundle("Value"=w50, "Value"=w49, "Value"=w48, "Value"=w47, "Value"=w17) -> (→"Table cluster_B":T41)  [unwired: 1 in]
  n198 = property on="Time Graph" class="XYGraph (strict)"(error in=w18) -> (error out=w294:errorcluster, "Value"=w285:cluster{"time":dbl[], "current":dbl[]}[])  [unwired: 1 in, 1 out]
  n199 = property on="CP Graph" class="XYGraph (strict)"(error in=w294) -> (error out=w293:errorcluster, "Value"=w284:cluster{i32[], dbl[]}[])  [unwired: 1 in, 1 out]
  n200 = property on="CP Graph Profile" class="XYGraph (strict)"(error in=w293) -> (error out=w292:errorcluster, "Value"=w283:cluster{i32[], dbl[]}[])  [unwired: 1 in, 1 out]
  n201 = property on="Time Graph Profile" class="XYGraph (strict)"(error in=w292) -> (error out=w291:errorcluster, "Value"=w297:cluster{"time":dbl[], dbl[]}[])  [unwired: 1 in, 1 out]
  n202 = property on="Signal Number Histogram" class="XYGraph (strict)"(error in=w291) -> (error out=w290:errorcluster, "Value"=w296:cluster{"配列 2":i32[], "配列 5":dbl[]}[])  [unwired: 1 in, 1 out]
  n203 = property on="Plot Graph" class="IntGraph (strict)"(error in=w290) -> (error out=w210:errorcluster, "Value"=w295:dbl[][])  [unwired: 1 in, 1 out]
  n204 = Bundle("Value"=w285, "Value"=w284, "Value"=w283, "Value"=w297, "Value"=w296, "Value"=w295) -> (→"GR data":T42)  [unwired: 1 in]
  n205 = case shown="True" w1 {
    tunnel: w210 -> [w367 w382]
    tunnel: [w367 w380] -> w169
    frame False {
    }
    frame True {
      n206 = property on="Base Ex Info" class="Clust (strict)"(error in=w382) -> (error out=w381:errorcluster, "Value"=w378:T17)  [unwired: 1 in, 1 out]
      n207 = property on="LSP Table" class="Tbl (strict)"(error in=w381) -> (error out=w387:errorcluster, "Value"=w392:string[][])  [unwired: 1 in, 1 out]
      n208 = property on="CP Profile Table" class="Tbl (strict)"(error in=w387) -> (error out=w386:errorcluster, "Value"=w391:string[][])  [unwired: 1 in, 1 out]
      n209 = property on="Time Profile Table" class="Tbl (strict)"(error in=w386) -> (error out=w385:errorcluster, "Value"=w390:string[][])  [unwired: 1 in, 1 out]
      n210 = property on="Signal Tag AZ" class="Arr (strict)"(error in=w385) -> (error out=w384:errorcluster, "Value"=w389:string[])  [unwired: 1 in, 1 out]
      n211 = property on="CP A Table Tag" class="Arr (strict)"(error in=w384) -> (error out=w372:errorcluster, "Value"=w388:string[])  [unwired: 1 in, 1 out]
      n212 = property on="Time A Table Tag" class="Arr (strict)"(error in=w372) -> (error out=w371:errorcluster, "Value"=w383:string[])  [unwired: 1 in, 1 out]
      n213 = property on="BNAL Path" class="Clust (strict)"(error in=w371) -> (error out=w370:errorcluster, "Value"=w376:T13)  [unwired: 1 in, 1 out]
      n214 = property on="Total assembly C" class="Clust (strict)"(error in=w370) -> (error out=w369:errorcluster, "Value"=w368:T6)  [unwired: 1 in, 1 out]
      n215 = property on="BC1" class="Clust (strict)"(error in=w369) -> (error out=w374:errorcluster, "Value"=w377:cluster{"B region#":i32, "Date":string})  [unwired: 1 in, 1 out]
      n216 = property on="LS Path" class="Clust (strict)"(error in=w374) -> (error out=w373:errorcluster, "Value"=w375:T14)  [unwired: 1 in, 1 out]
      n217 = Bundle("Value"=w392, "Value"=w391, "Value"=w390, "Value"=w389, "Value"=w388, "Value"=w383) -> (w379:T43)  [unwired: 1 in]
      "Save CV" <- w379
      n218 = call "BSM Signal Table Save.vi"("Base Ex Info"=w378, "Total assembly C"=w368, "BNAL Path"=w376, "error in"=w373, "Save CV"=w379, "BC1"=w377, "LS Path"=w375) -> ("error out"=w380:errorcluster)  [unwired: 4 in]
    }
  }
  "error out" <- w169
